vi "DropVI_SimpleClientSubscriber.vi"() -> ()   [LabVIEW 2013, in "MQTT Client.lvlib"]
uses:
  MQTT Client.lvlib
  Client class/Client.lvclass/Client.ctl
  <vilib>/LabVIEW Open Source Project/MQTT Connection/MQTT_Base/Base Class/MQTT_Base.lvclass/MQTT_Base.ctl
  <vilib>/LabVIEW Open Source Project/MQTT Control Packets/Control Packets/PUBLISH/PUBLISH.lvclass
  Client class/Client.lvclass
  <vilib>/LabVIEW Open Source Project/MQTT Connection/MQTT_Base/Base Class/MQTT_Base.lvclass
  <vilib>/LabVIEW Open Source Project/Connection/Connection/Connection.lvclass
  <vilib>/LabVIEW Open Source Project/Connection/Connection.TCP/Connection.TCP.lvclass
  <vilib>/LabVIEW Open Source Project/Connection/Connection.LocalQueue/Connection.LocalQueue.lvclass
panel:
  out "last error":errorcluster
  out "Unsuback":bool
  in  "Subscribe":bool
  in  "Connection":bool
  out "Waveform Chart":dbl(graph)
  out "Suback":bool
  in  "Stop Client":bool
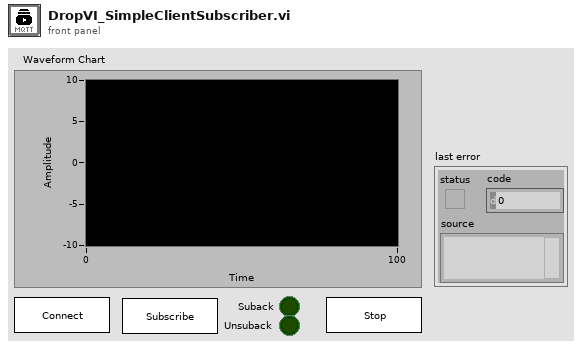
[diagram p1: front panel]
types:
  T1 = typedef "MQTT Client.lvlib/Client.lvclass/Public Events -- cluster.ctl" = cluster{"Connection Status":refnum<user-event>, "Connected":refnum<user-event>, "Application Message":refnum<user-event>}
  T2 = typedef "MQTT Base.lvlib/MQTT_Base.lvclass/Public Events -- cluster.ctl" = cluster{"Stop Event":refnum<user-event>, "Error Event":refnum<user-event>, "Inbound Message":refnum<user-event>}
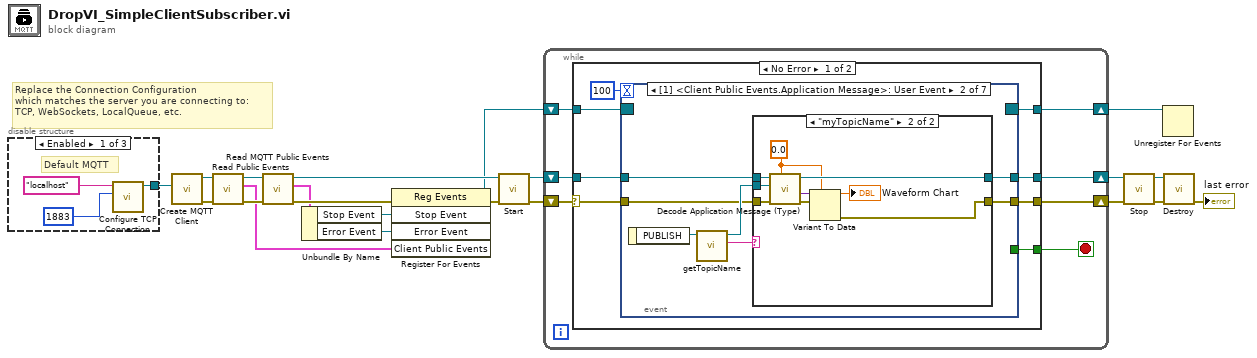
[diagram p0: block diagram]
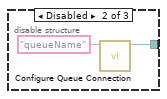
[diagram p2: hidden frame]
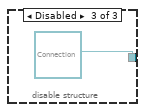
[diagram p3: hidden frame]
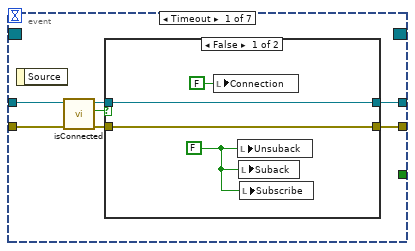
[diagram p4: hidden frame]
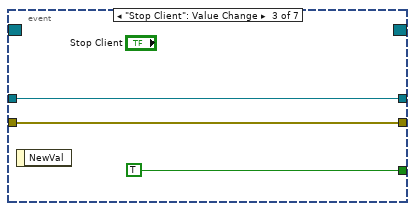
[diagram p7: hidden frame]
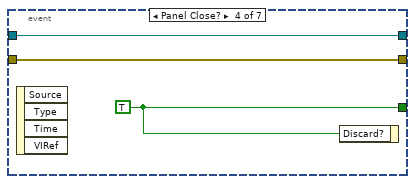
[diagram p8: hidden frame]
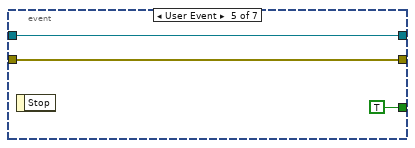
[diagram p9: hidden frame]
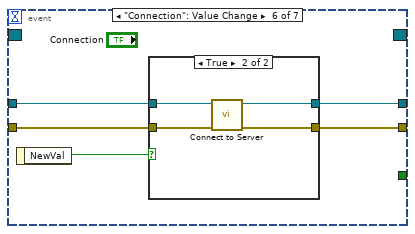
[diagram p10: hidden frame]
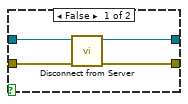
[diagram p11: hidden frame]
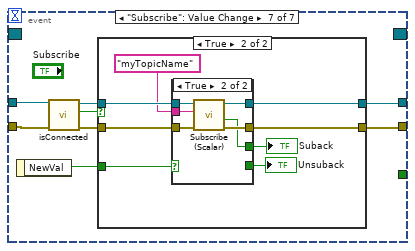
[diagram p12: hidden frame]
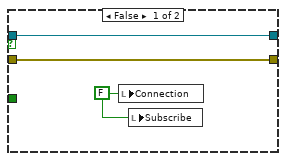
[diagram p13: hidden frame]
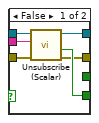
[diagram p14: hidden frame]
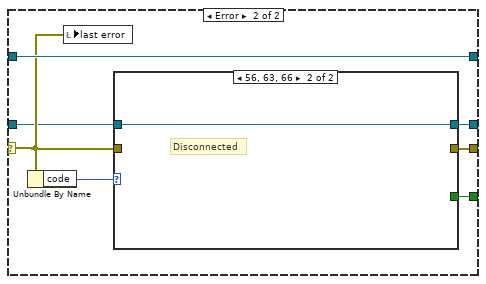
[diagram p15: hidden frame]
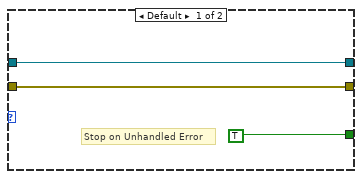
[diagram p16: hidden frame]
diagram:
  # "Replace the Connection Configuration\nwhich matches the server you are connecting to:\nTCP, WebSockets, LocalQueue, etc."
  n1 = disable-structure shown="Enabled" {
    disable-tunnel: [w23 w26 refnum<class "Connection.lvclass"> refnum ("Connection Configuration")] -> w1
    frame Enabled {
      # "Default MQTT"
      n2 = call <vilib>:"Configure TCP Connection.vi"("remote port (80)"=u16 1883, "address (localhost)"="localhost") -> ("Connection.TCP"=w23:refnum<class "Connection.TCP.lvclass">)  [unwired: 8 in, 1 out]
    }
    frame Disabled {
      n3 = call <vilib>:"Configure Queue Connection.vi"("Queue Name"="queueName") -> ("Connection.LocalQueue"=w26:refnum<class "Connection.LocalQueue.lvclass">)  [unwired: 9 in, 1 out]
    }
    frame Disabled {
    }
  }
  n4 = call "Create MQTT Client.vi"("Connection Configuration"=w1) -> ("error out"=w19:errorcluster, "Client out"=w21:refnum<class "Client.lvclass">)  [unwired: 9 in]
  n5 = call "Read Public Events.vi"("error in (no error)"=w19, "Client in"=w21) -> ("error out"=w18:errorcluster, "Client Public Events"=w16:T1, "Client out"=w20:refnum<class "Client.lvclass">)  [unwired: 7 in]
  n6 = call <vilib>:"Read MQTT Public Events.vi"("error in (no error)"=w18, "MQTT_Base in"=w20) -> ("error out"=w17:errorcluster, "MQTT Public Events"=w9:T2, "MQTT_Base out"=w14:refnum<class "Client.lvclass">)  [unwired: 7 in]
  n7 = Unbundle By Name(w9) -> ("Stop Event"=w11:refnum<user-event>, "Error Event"=w10:refnum<user-event>)
  n8 = register-events(error in=w17, w11, w10, w16) -> (reference out=w13:refnum<event-registration>, error out=w15:errorcluster)  [unwired: 1 in]
  n9 = call <vilib>:"Start.vi"("error in (no error)"=w15, "MQTT_Base in"=w14) -> ("error out"=w3:errorcluster, "MQTT_Base out"=w4:refnum<class "Client.lvclass">)  [unwired: 7 in, 1 out]
  n10 = while {
    shift-right: [w33] -> w12
    shift-left: w13 -> [w34]
    shift-right: [w30] -> w7
    shift-left: w4 -> [w31]
    shift-right: [w32] -> w5
    shift-left: w3 -> [w28]
    stop <- w29 stop-if-true
    n11 = case shown="No Error" w28 {
      selector: w28 -> [w35 w130]
      tunnel: w34 -> [w42 w133]
      tunnel: [w41 w133] -> w33
      tunnel: [w40 w128] -> w32
      tunnel: w31 -> [w38 w129]
      tunnel: [w37 w132] -> w30
      tunnel: [w36 w127] -> w29
      frame No Error {
        n12 = event shown="[1] <Client Public Events.Application Message>: User Event" {
          selector: w42 -> [_ _ _ _ _ _ _]
          dyn-events: [_ _ _ _ _ _ _] -> w41
          timeout: 100 -> [_ _ _ _ _ _ _]
          tunnel: w35 -> [w45 w59 w75 w77 w82 w83 w101]
          tunnel: [w48 w56 w75 w77 w82 w84 w102] -> w40
          tunnel: [_ _ TRUE w79 TRUE _ _] -> w36
          tunnel: w38 -> [w47 w60 w76 w78 w80 w87 w100]
          tunnel: [w49 w58 w76 w78 w80 w85 w103] -> w37
          event Timeout {
            n13 = event-data() -> ()  [unwired: 1 in, 1 out]
            n14 = call "isConnected.vi"("error in (no error)"=w45, "Client in"=w47) -> ("error out"=w44:errorcluster, "connected"=w43:bool, "Client out"=w46:refnum<class "Client.lvclass">)  [unwired: 7 in]
            n15 = case shown="False" w43 {
              tunnel: [w53 w55] -> w49
              tunnel: [w52 w54] -> w48
              tunnel: w46 -> [w53 w55]
              tunnel: w44 -> [w52 w54]
              frame False {
                w51 = FALSE
                n16 = local write "Connection"(FALSE ("Connection")) -> ()
                n17 = local write "Unsuback"(w51) -> ()
                n18 = local write "Suback"(w51) -> ()
                n19 = local write "Subscribe"(w51) -> ()
              }
              frame True {
              }
            }
          }
          event User Event {
            n20 = event-data() -> ("PUBLISH"=w62:refnum<class "PUBLISH.lvclass">)  [unwired: 1 in]
            n21 = call <vilib>:"getTopicName.vi"("PUBLISH in"=w62) -> ("Topic"=w57:string, "PUBLISH out"=w61:refnum<class "PUBLISH.lvclass">)  [unwired: 8 in, 1 out]
            n22 = case shown="\"myTopicName\"" w57 {
              tunnel: w61 -> [_ w65]
              tunnel: w60 -> [w64 w71]
              tunnel: w59 -> [w63 w69]
              tunnel: [w64 w70] -> w58
              tunnel: [w63 w73] -> w56
              frame Default {
              }
              frame "myTopicName" {
                w67 = 0.0
                n23 = call "Decode Application Message (Type).vi"("Type"=w67, "error in (no error)"=w69, "PUBLISH"=w65, "Client in"=w71) -> ("error out"=w68:errorcluster, "Payload"=w66:variant, "Client out"=w70:refnum<class "Client.lvclass">)  [unwired: 4 in, 1 out]
                n24 = Variant To Data(error in=w68, type=w67, Variant=w66) -> (data=→"Waveform Chart":dbl, error out=w73:errorcluster)
              }
            }
          }
          event "Stop Client": Value Change {
            n25 = event-data() -> ()  [unwired: 1 in, 1 out]
          }
          event Panel Close? {
            w79 = TRUE
            n26 = event-data() -> ()  [unwired: 1 in, 4 out]
            n27 = event-data("Discard?"=w79) -> ()  [unwired: 1 in, 1 out]
          }
          event User Event {
            n28 = event-data() -> ()  [unwired: 1 in, 1 out]
          }
          event "Connection": Value Change {
            n29 = event-data() -> ("NewVal"=w86:bool)  [unwired: 1 in]
            n30 = case shown="True" w86 {
              tunnel: w87 -> [w91 w95]
              tunnel: [w90 w92] -> w85
              tunnel: [w89 w93] -> w84
              tunnel: w83 -> [w88 w94]
              frame False {
                n31 = call "Disconnect from Server.vi"("error in (no error)"=w88, "Client in"=w91) -> ("error out"=w89:errorcluster, "Client out"=w90:refnum<class "Client.lvclass">)  [unwired: 7 in, 1 out]
              }
              frame True {
                n32 = call "Connect to Server.vi"("error in (no error)"=w94, "Client in"=w95) -> ("error out"=w93:errorcluster, "Client out"=w92:refnum<class "Client.lvclass">)  [unwired: 6 in, 2 out]
              }
            }
          }
          event "Subscribe": Value Change {
            n33 = event-data() -> ("NewVal"=w96:bool)  [unwired: 1 in]
            n34 = call "isConnected.vi"("error in (no error)"=w101, "Client in"=w100) -> ("error out"=w98:errorcluster, "connected"=w97:bool, "Client out"=w99:refnum<class "Client.lvclass">)  [unwired: 7 in]
            n35 = case shown="True" w97 {
              tunnel: [w106 w114] -> w103
              tunnel: [w105 w113] -> w102
              tunnel: w99 -> [w106 w112]
              tunnel: w98 -> [w105 w111]
              tunnel: w96 -> [_ w109]
              frame False {
                w104 = FALSE ("Connection")
                n36 = local write "Connection"(w104) -> ()
                n37 = local write "Subscribe"(w104) -> ()
              }
              frame True {
                n38 = case shown="True" w109 {
                  tunnel: [w115 w123] -> w114
                  tunnel: [w116 w122] -> w113
                  tunnel: w112 -> [w120 w126]
                  tunnel: w111 -> [w119 w125]
                  tunnel: "myTopicName" ("Topic Name (empty: Payload name)") -> [w118 w124]
                  tunnel: [_ w121] -> w108
                  tunnel: [w117 _] -> w107
                  frame False {
                    n39 = call "Unsubscribe (Scalar).vi"("error in (no error)"=w119, "Topic Filter"=w118, "Client in"=w120) -> ("error out"=w116:errorcluster, "Ack"=w117:bool, "Client out"=w115:refnum<class "Client.lvclass">)  [unwired: 6 in]
                  }
                  frame True {
                    n40 = call "Subscribe (Scalar).vi"("error in (no error)"=w125, "Topic Filter"=w124, "Client in"=w126) -> ("error out"=w122:errorcluster, "Ack"=w121:bool, "Client out"=w123:refnum<class "Client.lvclass">)  [unwired: 6 in]
                  }
                }
                "Unsuback" <- w107
                "Suback" <- w108
              }
            }
          }
        }
      }
      frame Error {
        n41 = Unbundle By Name(w130) -> ("code"=w131:i32)
        n42 = local write "last error"(w130) -> ()
        n43 = case shown="56, 63, 66" w131 {
          tunnel: w129 -> [w136 w137]
          tunnel: [w136 w137] -> w132
          tunnel: w130 -> [w135 _]
          tunnel: [w135 _] -> w128
          tunnel: [TRUE _] -> w127
          frame Default {
            # "Stop on Unhandled Error"
          }
          frame 56, 63, 66 {
            # "Disconnected"
          }
        }
      }
    }
  }
  n44 = call <vilib>:"Stop.vi"("error in (no error)"=w5, "MQTT_Base in"=w7) -> ("error out"=w6:errorcluster, "MQTT_Base out"=w8:refnum<class "Client.lvclass">)  [unwired: 7 in, 1 out]
  n45 = Unregister For Events(event registration refnum=w12) -> ()  [unwired: 1 in, 1 out]
  n46 = call <vilib>:"Destroy.vi"("error in (no error)"=w6, "MQTT_Base in"=w8) -> ("error out"=→"last error":errorcluster)  [unwired: 8 in, 1 out]
